vi "Mspec Stitcher gui.vi"() -> ()   [LabVIEW 2020]
uses:
  Shared/GUI_Template/GUI_master/tcp_new_data_event.ctl
  Shared/GUI_Template/GUI_master/tcp new data cluster.ctl
  <vilib>/ErrorRing/Error Ring.xnode
panel:
  out "error img to array":errorcluster
  out "stitched array image":u16[][](graph)
  in  "MinE::1":dbl caption="MinE" min=0.0 max=0.0
  in  "MinAngle::1":dbl caption="MinAngle" min=0.0 max=0.0
  in  "DeltaAngle::1":dbl caption="DeltaAngle" min=0.0 max=0.0
  in  "DeltaE::1":dbl caption="DeltaE" min=0.0 max=0.0
  in  "GUIdevice 1":string="ANALY-TEA-MagSpecSticher" caption="CAMERA 1"
  out "image::1":T1(plugin-control) caption="M1 Cam"
  out "tcp data event":T2
  in  "stop":bool
  out "error IO 2":errorcluster
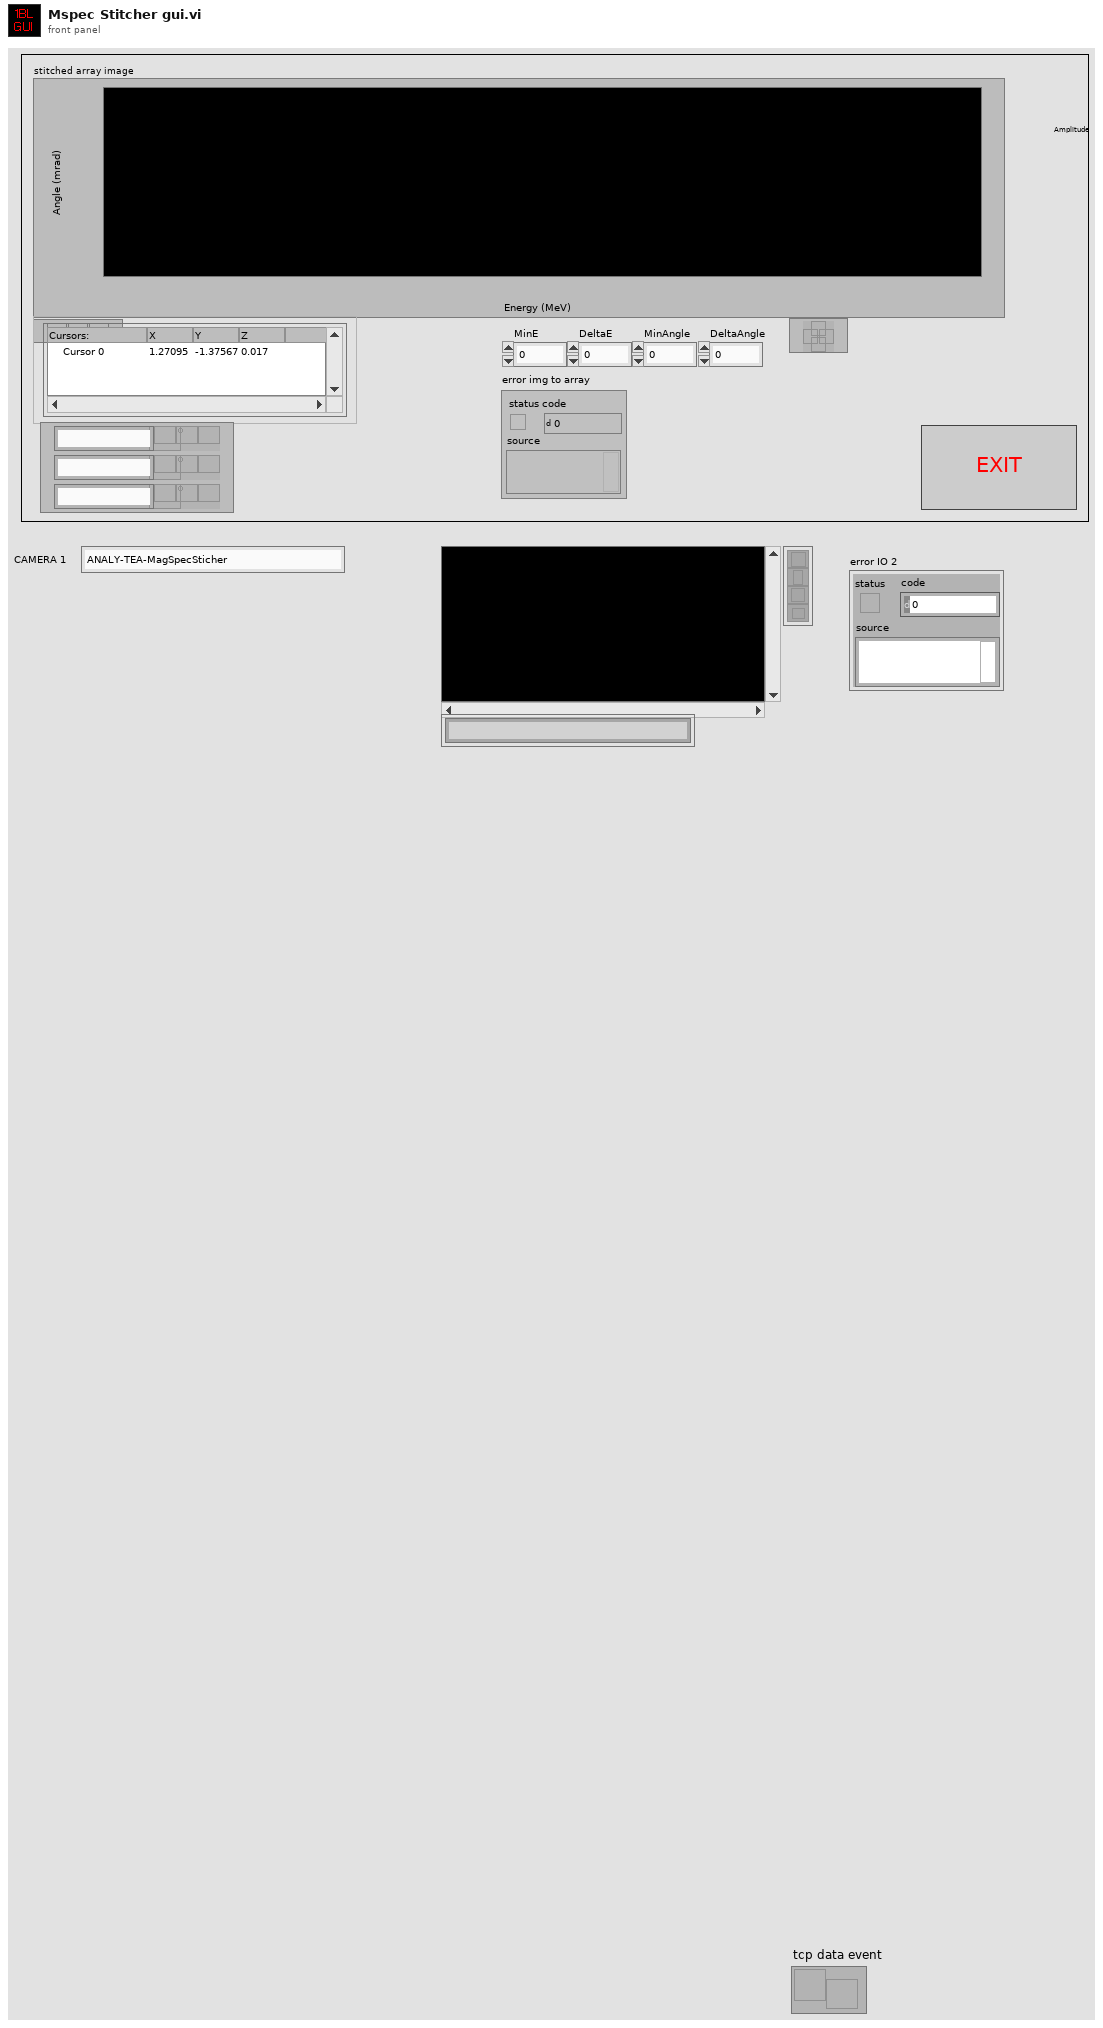
[diagram p1: front panel]
types:
  T1 = typedef "IMAQ Image.ctl" = refnum<image>
  T2 = typedef "tcp_new_data_event.ctl" = refnum<user-event>
  T3 = cluster{"Last update Cam1":u32, "Last update Cam2":u32, "Last update Cam3":u32, "Last update Cam4":u32, "Last update Cam5":u32, "Last update Cam6":u32, "Last update Cam7":u32, "Last update Cam8":u32}
  T4 = typedef "Image Type" = u32
  T5 = typedef "tcp new data cluster.ctl" = cluster{"EventEnum":enum16{"new data", "connection status update"}, "Device name":string}
  T6 = enum32{"invalid app kind", "Development System", "Run Time System", "Student Edition", "Embedded LabVIEW", "Evaluation", "Custom"}
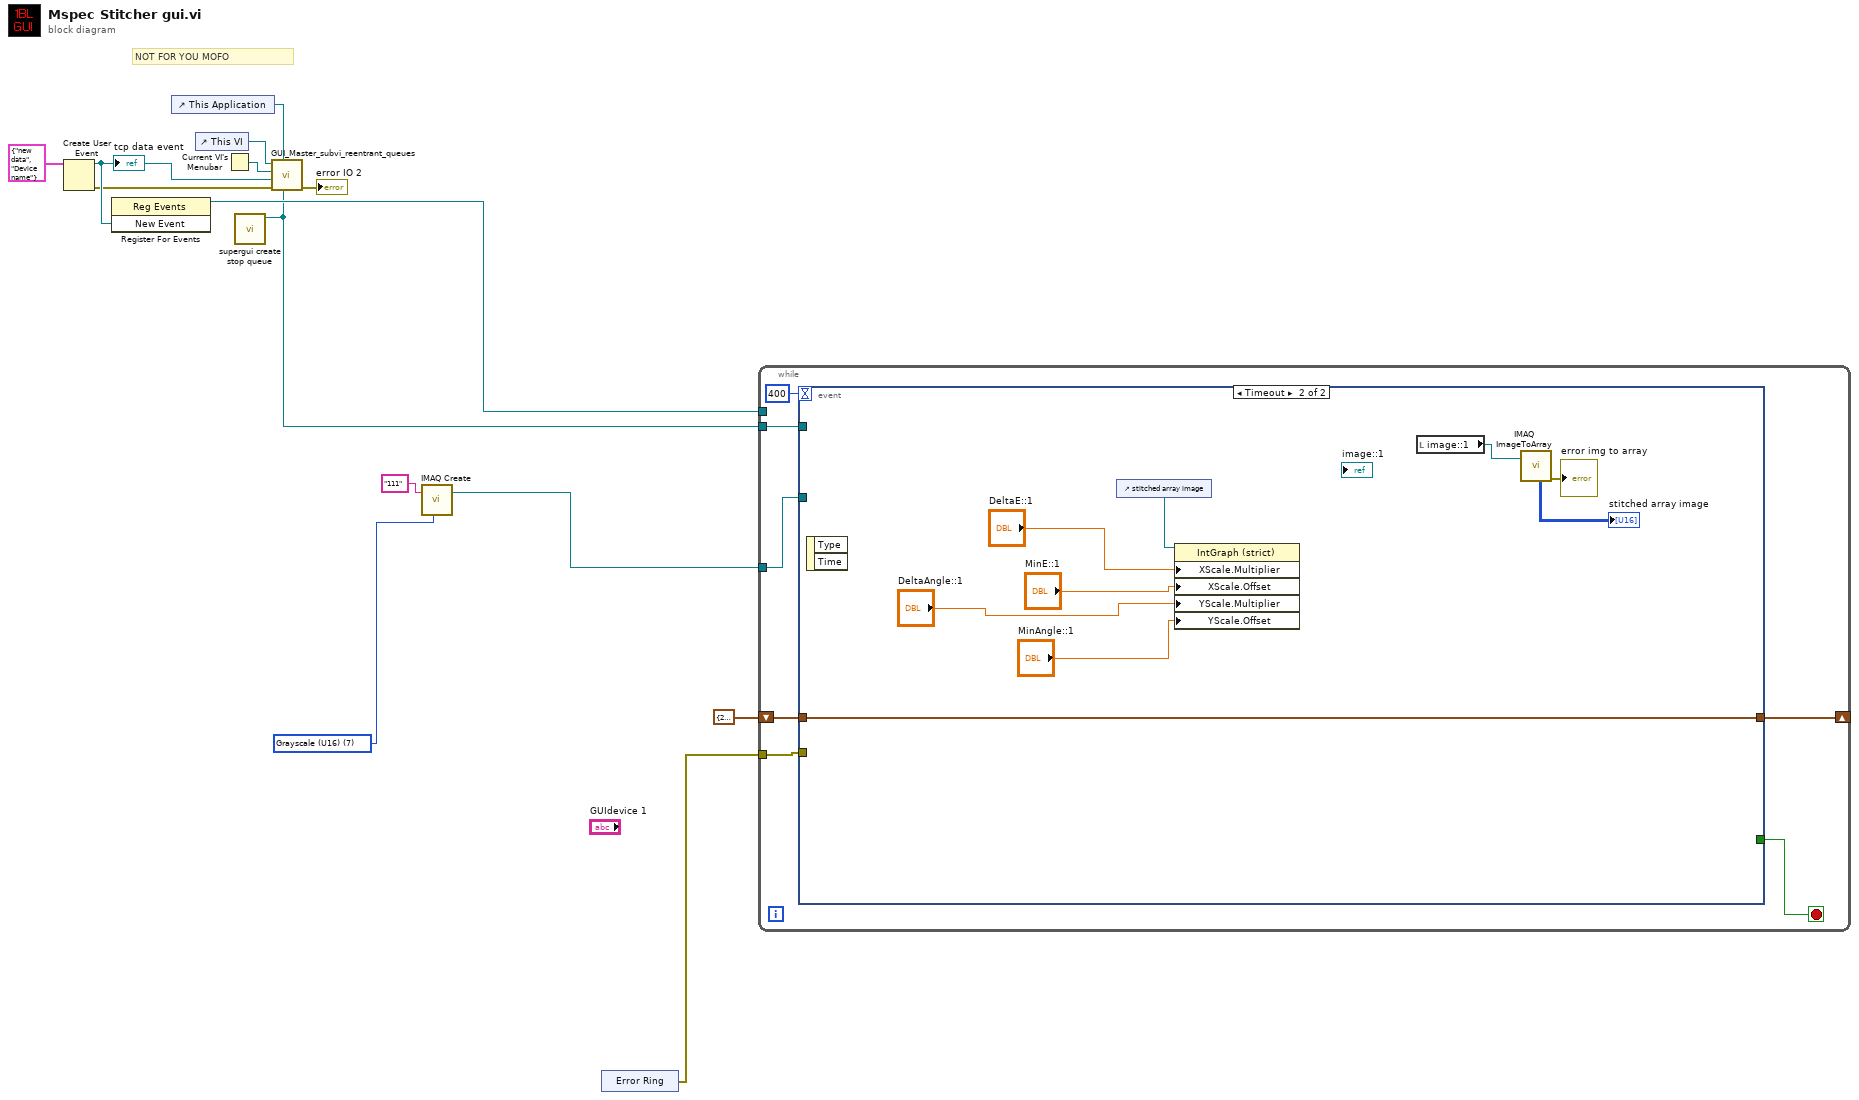
[diagram p0: block diagram]
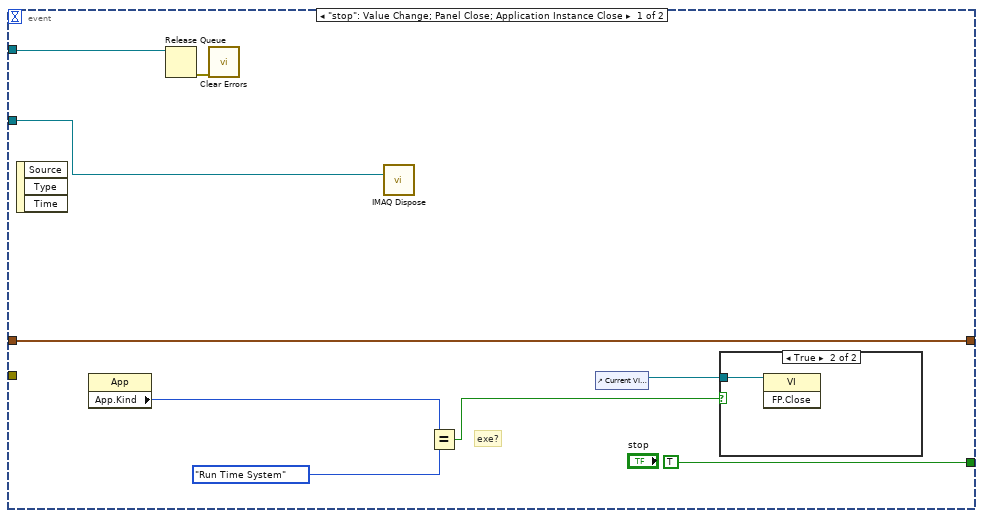
[diagram p2: hidden frame]
diagram:
  w1 = T4 7 items=["Grayscale (U8)", "Grayscale (I16)", "Grayscale (SGL)", "Complex (CSG)", "RGB (U32)", "HSL (U32)", "RGB (U64)", "Grayscale (U16)"] ("Image Type")
  # "NOT FOR YOU MOFO"
  n1 = Create User Event(user event datatype=T5 {"EventEnum"=enum."new data", "Device name"="Device name"} ("New Event")) -> (user event=w13:refnum<user-event>, error out=w12:errorcluster)  [unwired: 1 in]
  "tcp data event" <- w13
  n2 = register-events(w13) -> (reference out=w8:refnum<event-registration>)  [unwired: 2 in, 1 out]
  n3 = control-ref of="This Application"() -> (w14:refnum<vi>)
  n4 = control-ref of="This VI"() -> (w9:refnum<vi>)
  n5 = Current VI's Menubar() -> (w10:refnum<k9>)
  n6 = call "supergui create stop queue.vi"() -> ("STOP Queue out"=w4:refnum<queue>)  [unwired: 11 in]
  n7 = call "GUI_Master_subvi_reentrant_queues.vi"("STOP Queue in"=w4, "This Application"=w14, "error in (no error)"=w12, "tcp data event"=w13, "Caller menu reference"=w10, "Caller VI ref"=w9) -> ("error out"=→"error IO 2":errorcluster)  [unwired: 5 in]
  n8 = call "IMAQ Create"("Image Name"="111", "Image Type"=w1) -> ("New Image"=w2:T1)  [unwired: 3 in, 1 out]
  n9 = xnode "Error Ring"() -> ("error out"=w3:errorcluster)
  n10 = while {
    tunnel: w8 -> [_]
    shift-right: [w19] -> _
    shift-left: T3 {"Last update Cam1"=200, "Last update Cam2"=200, "Last update Cam3"=200, "Last update Cam4"=200, "Last update Cam5"=200, "Last update Cam6"=200, "Last update Cam7"=200, "Last update Cam8"=200} -> [w20]
    tunnel: w4 -> [w18]
    tunnel: w2 -> [w17]
    tunnel: w3 -> [w16]
    stop <- w21 stop-if-true
    n11 = event shown="[1] Timeout" {
      selector: _ -> [_ _]
      dyn-events: _ -> [_ _]
      timeout: 400 -> [_ _]
      tunnel: [TRUE ("stop") _] -> w21
      tunnel: w20 -> [w29 w40]
      tunnel: [w29 w40] -> w19
      tunnel: w18 -> [w28 _]
      tunnel: w17 -> [w26 _]
      tunnel: w16 -> [_ _]
      event "stop": Value Change; Panel Close; Application Instance Close {
        # "exe?"
        n12 = event-data() -> ()  [unwired: 1 in, 3 out]
        n13 = property class="App"() -> ("App.Kind"=w24:T6)  [unwired: 2 in, 2 out]
        n14 = Release Queue(queue=w28) -> (error out=w27:errorcluster)  [unwired: 2 in, 2 out]
        n15 = call <vilib>:"Clear Errors.vi"("error in (no error)"=w27) -> ()  [unwired: 5 in, 2 out]
        n16 = call "IMAQ Dispose"("Image"=w26) -> ()  [unwired: 5 in, 1 out]
        n17 = Equal?(x=w24, y=T6."Run Time System" ("Application:Kind")) -> (x = y?=w22:bool)
        n18 = control-ref of="Current VI Reference"() -> (w25:refnum<vi>)
        n19 = case shown="True" w22 {
          tunnel: w25 -> [_ w31]
          frame False {
          }
          frame True {
            n20 = invoke class="VI" method="FP.Close"(reference=w31) -> ()  [unwired: 2 in, 3 out]
          }
        }
      }
      event Timeout {
        n21 = event-data() -> ()  [unwired: 1 in, 2 out]
        n22 = control-ref of="stitched array image"() -> (w35:refnum<vi>)
        n23 = property on="Property Node" class="IntGraph (strict)"(reference=w35, "XScale.Multiplier"="DeltaE::1", "XScale.Offset"="MinE::1", "YScale.Multiplier"="DeltaAngle::1", "YScale.Offset"="MinAngle::1") -> ()  [unwired: 1 in, 2 out]
        n24 = local read "image::1"() -> (w33:T1)
        n25 = call "IMAQ ImageToArray"("Image"=w33) -> ("Image Pixels (U16)"=→"stitched array image":u16[][], "error out"=→"error img to array":errorcluster)  [unwired: 3 in, 3 out]
      }
    }
  }
